vi "Check Connection.vi"(8 "error in (no error)":errorcluster, 11 "Plugin in":refnum<class "Modbus.lvclass">) -> (0 "error out":errorcluster, 3 "Plugin out":refnum<class "Modbus.lvclass">)   [LabVIEW 2026, in "Modbus.lvlib" / "Modbus.lvclass"]
uses:
  Modbus.lvclass
  Modbus.lvclass/Modbus.ctl
  <vilib>/ni/Modbus Library/API/Master/Modbus Master.lvclass
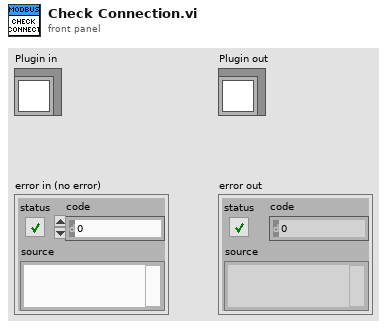
[diagram p1: front panel]
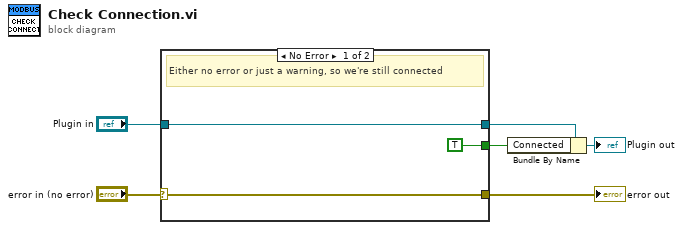
[diagram p0: block diagram]
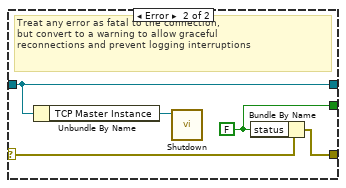
[diagram p2: hidden frame]
diagram:
  n1 = case shown="No Error" "error in (no error)" {
    selector: "error in (no error)" -> [w9 w14]
    tunnel: [w9 w13] -> w5
    tunnel: [TRUE w10] -> w1
    tunnel: "Plugin in" -> [w7 w12]
    tunnel: [w7 w12] -> w3
    frame No Error {
      # "Either no error or just a warning, so we're still connected"
    }
    frame Error {
      w10 = FALSE ("status")
      # "Treat any error as fatal to the connection,\nbut convert to a warning to allow graceful\nreconnections and prevent logging interruptions"
      n2 = Unbundle By Name(w12) -> ("TCP Master Instance"=w11:refnum<class "Modbus Master.lvclass">)
      n3 = call-dynamic "Shutdown.vi"("Modbus master in"=w11) -> ()  [unwired: 10 in, 1 out]
      n4 = Bundle By Name(cluster=w14, "status"=w10) -> (w13:errorcluster)
    }
  }
  "error out" <- w5
  n5 = Bundle By Name(cluster=w3, "Connected"=w1) -> (→"Plugin out":refnum<class "Modbus.lvclass">)
